vi "Throw Async Handler Error.vi"(8 "error in (no error)":errorcluster, 10 "Error":errorcluster, 11 "Mock Async Handler Process in":refnum<class "Mock Async Handler Process.lvclass">) -> (0 "error out":errorcluster, 3 "Mock Async Handler Process out":refnum<class "Mock Async Handler Process.lvclass">)   [LabVIEW 2020, in "Mock Async Handler Process.lvclass"]
uses:
  Mock Async Handler Process.lvclass
  Mock Async Handler Process.lvclass/Mock Async Handler Process.ctl
  source/Framework/Process/Process.lvclass
  C:/git/astemes-triarc-framework/source/Framework/Process/Process.lvclass
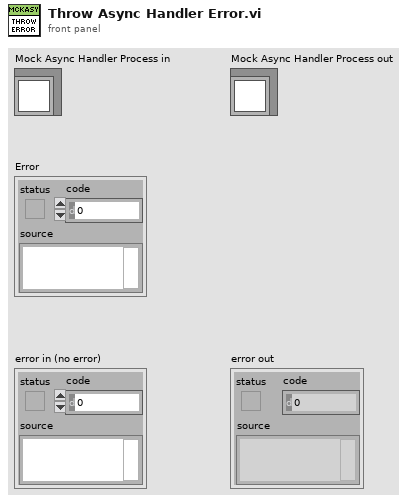
[diagram p1: front panel]
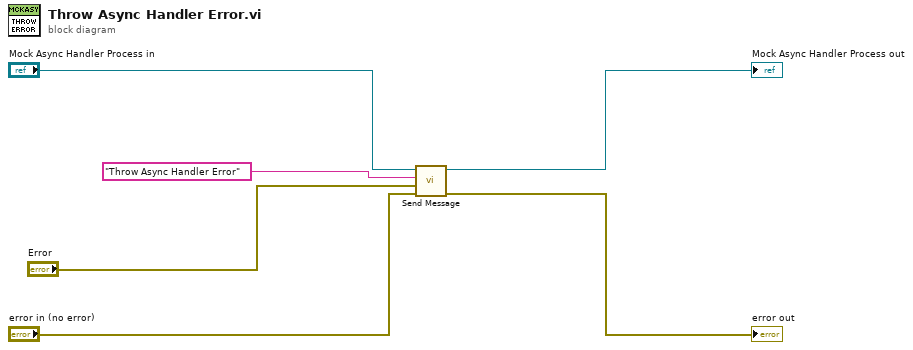
[diagram p0: block diagram]
diagram:
  n1 = call "Send Message.vi"("error in (no error)"="error in (no error)", "Message Data"="Error", "Message"="Throw Async Handler Error", "Process In"="Mock Async Handler Process in") -> ("error out"=→"error out":errorcluster, "Process Out"=→"Mock Async Handler Process out":refnum<class "Mock Async Handler Process.lvclass">)  [unwired: 6 in]
